vi "Write file.vi"(8 "error in (no error)":errorcluster, 11 "Graph data":T1) -> (0 "error out":errorcluster)   [LabVIEW 2020]
uses:
  controls/Graph data --typedef.ctl
  <vilib>/Utility/sysdir.llb/System Directory Type.ctl
  <vilib>/Utility/file.llb/Write Delimited Spreadsheet (string).vi
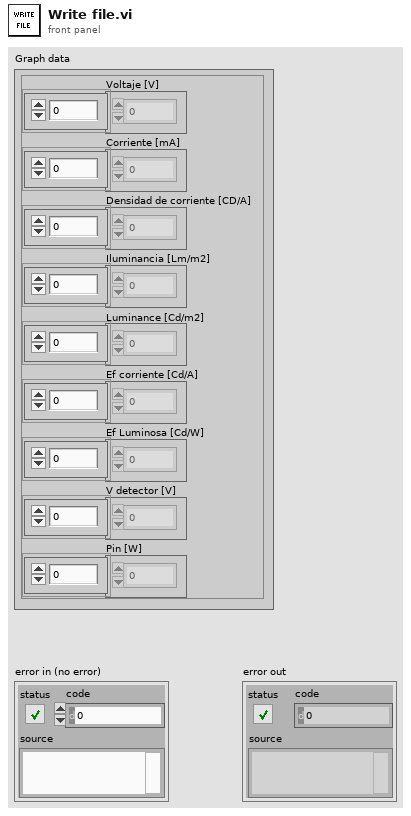
[diagram p1: front panel]
types:
  T1 = typedef "Graph data --typedef.ctl" = cluster{"Voltaje [V]":dbl[], "Corriente [mA]":dbl[], "Densidad de corriente [CD/A]":dbl[], "Iluminancia [Lm/m2]":dbl[], "Luminance [Cd/m2]":dbl[], "Ef corriente [Cd/A]":dbl[], "Ef Luminosa [Cd/W]":dbl[], "V detector [V]":dbl[], "Pin [W]":dbl[]}
  T2 = typedef "System Directory Type.ctl" = i32
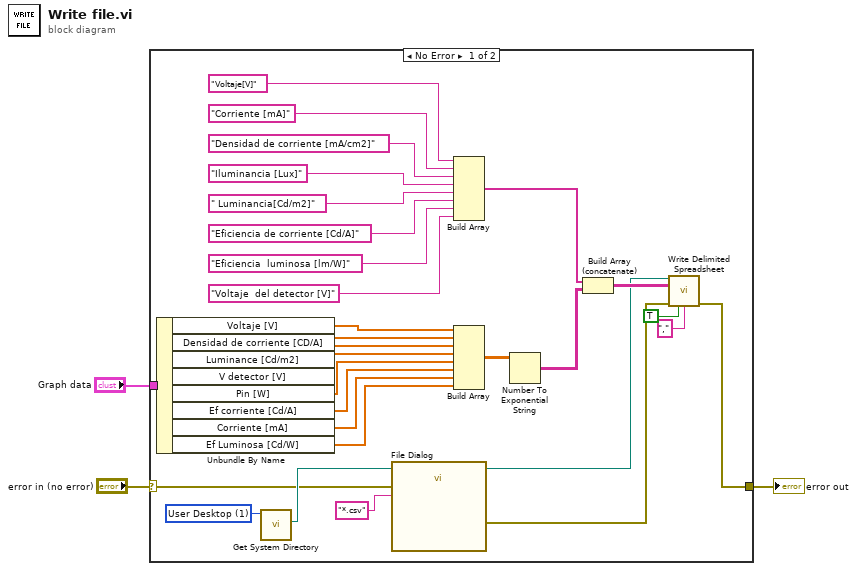
[diagram p0: block diagram]
diagram:
  n1 = case shown="No Error" "error in (no error)" {
    selector: "error in (no error)" -> [w8 w34]
    tunnel: "Graph data" -> [w29 _]
    tunnel: [w12 w34] -> w2
    frame No Error {
      w11 = T2 1 items=["User Home"=0, "User Desktop"=1, "User Documents"=2, "User Application Data"=3, "User Preferences"=4, "User Temporary"=5, "Public Documents"=6, "Public Application Data"=7, "Public Preferences"=8, "Public Cache"=13, "System Core Libraries"=9, "System Installed Libraries"=10, "Application Files"=11, "Boot Volume Root"=12] ("system directory type")
      n2 = Unbundle By Name(w29) -> ("Voltaje [V]"=w30:dbl[], "Densidad de corriente [CD/A]"=w31:dbl[], "Luminance [Cd/m2]"=w32:dbl[], "V detector [V]"=w33:dbl[], "Pin [W]"=w20:dbl[], "Ef corriente [Cd/A]"=w19:dbl[], "Corriente [mA]"=w18:dbl[], "Ef Luminosa [Cd/W]"=w17:dbl[])
      n3 = call <vilib>:"Get System Directory.vi"("system directory type"=w11) -> ("system directory"=w10:path)  [unwired: 10 in]
      n4 = call "File Dialog"("start path"=w10, "error in"=w8, "pattern (all files)"="*.csv") -> ("selected path"=w9:path, "error out"=w6:errorcluster)  [unwired: 9 in, 2 out]
      n5 = Build Array("Voltaje[V]", "Corriente [mA]", "Densidad de corriente [mA/cm2]", "Iluminancia [Lux]", " Luminancia[Cd/m2]", "Eficiencia de corriente [Cd/A]", "Eficiencia  luminosa [lm/W]", "Voltaje  del detector [V]") -> (w15:string[])
      n6 = Build Array(w30, w31, w32, w33, w20, w19, w18, w17) -> (w16:dbl[][])
      n7 = Number To Exponential String(number=w16) -> (E-format string=w14:string[][])  [unwired: 1 in, 2 out]
      n8 = Build Array (concatenate)(w15, w14) -> (w13:string[][])
      n9 = call-poly <vilib>:"Write Delimited Spreadsheet.vi"("file path (dialog if empty)"=w9, "2D data"=w13, "error in (no error)"=w6, "transpose? (no:F)"=TRUE, "delimiter (\\t)"="," ("delimiter (\\t)")) -> ("error out"=w12:errorcluster)  [unwired: 9 in, 1 out]
    }
    frame Error {
    }
  }
  "error out" <- w2
